vi "libssh2_channel_eof.vi"(8 "error in (no error)":errorcluster, 11 "channel":T1) -> (0 "error out":errorcluster, 2 "eof":bool)   [LabVIEW 2017, in "libssh2.lvlib"]
doc: "Check the EOF status of the channel."
uses:
  libssh2.lvlib
  Channel Refnum.ctl
  Acquire Session.vi
  Release Session.vi
  Not A Channel.vi
  <vilib>/Utility/error.llb/Error Cluster From Error Code.vi
  Global Settings.vi
  Read Channel Refnum.vi
  Read Session Refnum.vi
  <vilib>/Utility/semaphor.llb/Acquire Semaphore.vi
  <vilib>/Utility/semaphor.llb/Release Semaphore.vi
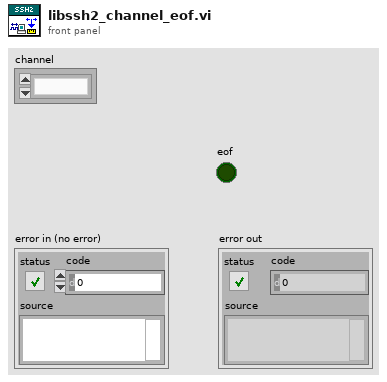
[diagram p1: front panel]
types:
  T1 = typedef "libssh2.lvlib/Channel Refnum.ctl" = refnum<k1>
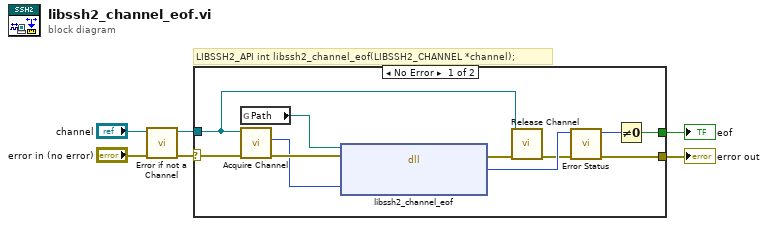
[diagram p0: block diagram]
diagram:
  # "LIBSSH2_API int libssh2_channel_eof(LIBSSH2_CHANNEL *channel);"
  n1 = call "Error if not a Channel.vi"("error in (no error)"="error in (no error)", "channel"="channel") -> ("error out"=w3:errorcluster, "channel out"=w1:T1)  [unwired: 8 in]
  n2 = case shown="No Error" w3 {
    selector: w3 -> [w17 w18]
    tunnel: [w16 w18] -> w6
    tunnel: w1 -> [w7 _]
    tunnel: [w15 _] -> w4
    frame No Error {
      n3 = global read "Global Settings.vi" "Path"() -> (w11:path)
      n4 = call "Acquire Channel.vi"("error in (no error)"=w17, "channel"=w7) -> ("error out"=w13:errorcluster, "LIBSSH2_CHANNEL*"=w12:u64)  [unwired: 8 in]
      n5 = dll-call lib="?" fn="libssh2_channel_eof"(path in=w11, error in=w13, "channel"=w12) -> (error out=w14:errorcluster, "return value"=w10:i32)  [unwired: 2 in, 1 out]
      n6 = call "Release Channel.vi"("error in (no error)"=w14, "channel"=w7) -> ("error out"=w8:errorcluster)  [unwired: 9 in]
      n7 = call "Error Status.vi"("error in (no error)"=w8, "return value"=w10) -> ("error out"=w16:errorcluster, "return value out"=w9:i32)  [unwired: 8 in]
      n8 = Not Equal To 0?(x=w9) -> (x != 0?=w15:bool)
    }
    frame Error {
    }
  }
  "error out" <- w6
  "eof" <- w4
